vi "Copy.vi"(8 "error in":errorcluster, 9 "Target Folder":path, 10 "Source File":path, 11 "IFile Manager in":refnum<class "Mock IFile Manager.lvclass">) -> (0 "error out":errorcluster, 2 "New Path":path, 3 "IFile Manager out":refnum<class "Mock IFile Manager.lvclass">)   [LabVIEW 2026, in "Mock IFile Manager.lvclass"]
doc: "This VI copies the specified source file to the target directory. If the target already exists it will be overwritten."
uses:
  Mock IFile Manager.lvclass
  C:/Program Files/National Instruments/LabVIEW 2026/vi.lib/Astemes/LMock/Mock.lvclass
  Mock IFile Manager.lvclass/Mock IFile Manager.ctl
  <vilib>/Astemes/LMock/Mock.lvclass
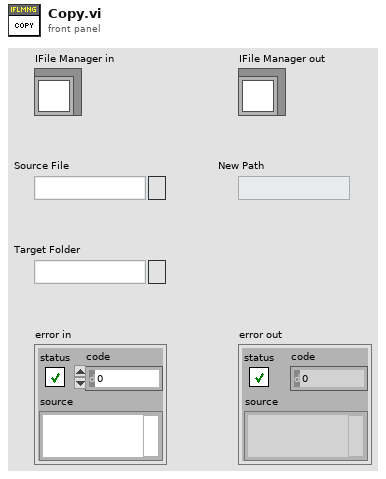
[diagram p1: front panel]
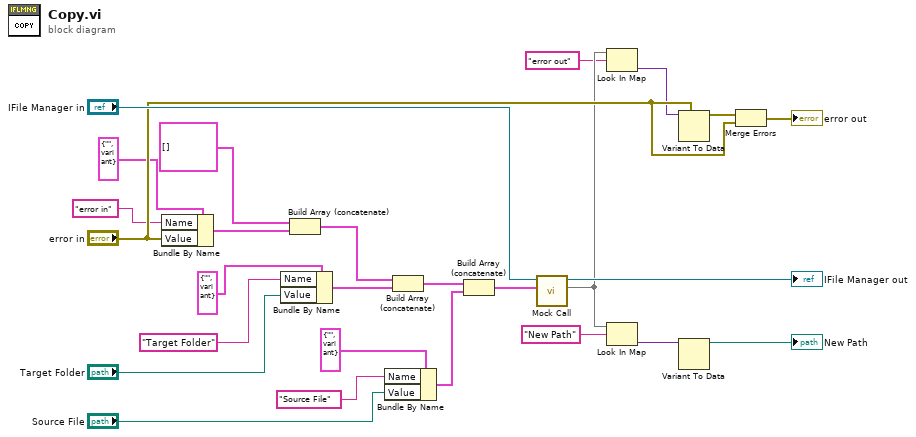
[diagram p0: block diagram]
diagram:
  n1 = Bundle By Name(cluster=cluster{"Name":string, "Value":variant} {"Name"="", "Value"=variant} ("element"), "Name"="error in", "Value"="error in") -> (w5:cluster{"Name":string, "Value":variant})
  n2 = Bundle By Name(cluster=cluster{"Name":string, "Value":variant} {"Name"="", "Value"=variant} ("element"), "Name"="Target Folder", "Value"="Target Folder") -> (w3:cluster{"Name":string, "Value":variant})
  n3 = Build Array (concatenate)(cluster{"Name":string, "Value":variant}[] [] ("Control Values"), w5) -> (w17:cluster{"Name":string, "Value":variant}[])
  n4 = Bundle By Name(cluster=cluster{"Name":string, "Value":variant} {"Name"="", "Value"=variant} ("element"), "Name"="Source File", "Value"="Source File") -> (w1:cluster{"Name":string, "Value":variant})
  n5 = Build Array (concatenate)(w17, w3) -> (w20:cluster{"Name":string, "Value":variant}[])
  n6 = Build Array (concatenate)(w20, w1) -> (w23:cluster{"Name":string, "Value":variant}[])
  n7 = call <vilib>:"Mock Call.vi"("Control Values"=w23, "Mock In"="IFile Manager in") -> ("Return Values"=w15:map{string, variant}, "Mock Out"=→"IFile Manager out":refnum<class "Mock IFile Manager.lvclass">)  [unwired: 8 in]
  n8 = Look In Map(map=w15, key="error out") -> (value=w10:variant)  [unwired: 1 in, 1 out]
  n9 = Look In Map(map=w15, key="New Path") -> (value=w13:variant)  [unwired: 1 in, 1 out]
  n10 = Variant To Data(type="error in", Variant=w10) -> (data=w9:errorcluster)  [unwired: 1 in, 1 out]
  n11 = Variant To Data(Variant=w13) -> (data=→"New Path":path)  [unwired: 2 in, 1 out]
  n12 = Merge Errors(w9, "error in") -> (→"error out":errorcluster)
